vi "Run.vi"(8 "error in (no error)":errorcluster, 10 "Timing Source":string, 11 "Audio Output Queue":refnum<queue>) -> (0 "error out":errorcluster)   [LabVIEW 2019, in "Audio Engine.lvlib"]
doc: "The main audio processing loop.\n\n<b>Priority:</b> Above Normal\n<b>Execution System:</b> Standard"
uses:
  Audio Engine.lvlib
  Audio Output/Audio Output Queue Type.ctl
  <vilib>/Platform/TimedLoop/XDataNode/timing_clust.ctl
  <vilib>/Platform/TimedLoop/XDataNode/nitl_modes.ctl
  <vilib>/Platform/TimedLoop/XDataNode/wakeup.ctl
  Packed Libraries/Globals.lvlibp/Constants.vi
  Packed Libraries/Audio Processing.lvlibp/DBL To I16.vi
  <vilib>/platform/TimedLoop/XDataNode/XDataNode.xnode
  Classes/Deck/Deck.lvclass
  Classes/Mixer/Mixer.lvclass
  <vilib>/Platform/TimedLoop/XDataNode/XDNodeRunTimeDep.lvlib
  Audio Output/Audio Output.lvlib
  Packed Libraries/Globals.lvlibp
  Classes/Effect Unit/Effect Unit.lvclass
  Classes/Channel/Channel.lvclass
  Packed Libraries/Messaging.lvlibp
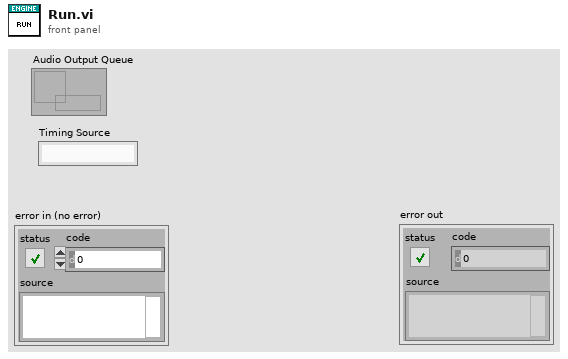
[diagram p1: front panel]
types:
  T1 = typedef "Audio Output.lvlib/Audio Output Queue Type.ctl" = cluster{"Master":waveform(i16)[], "Headphones":waveform(i16)[], "Start Time":dbl}
  T2 = typedef "XDNodeRunTimeDep.lvlib/timing_clust.ctl" = cluster{"Expected End [f-1]":u64, "Actual End [f-1]":u64, "Finished Late? [f-1]":bool, "Expected End [i-1]":u64, "Actual End [i-1]":u64, "Finished Late? [i-1]":bool, "Expected Start [i]":u64, "Actual Start [i]":u64, "Expected Start [f]":u64, "Actual Start [f]":u64, "Source Name":string, "Structure Name":string, "Period":i64, "Deadline":i64, "Offset":i64, "Start":i64, "Priority":i32, "Timeout":i32, "Mode":T3, "Wakeup Reason":T4, "Error":errorcluster, "Source Type":string, "Secondary Source Type":string, "Global End Time":u64, "Global Start Time":u64, "Frame Duration":u64, "Iteration Duration":u64, "Assigned CPU":i32, "I/O Scan Engine Mode":u32}
  T3 = typedef "XDNodeRunTimeDep.lvlib/nitl_modes.ctl" = enum32{"No Change", "Process missed periods, maintain original phase", "Discard missed periods, maintain original phase", "Process missed periods, ignore original phase", "Discard missed periods, ignore original phase"}
  T4 = typedef "XDNodeRunTimeDep.lvlib/wakeup.ctl" = enum32{"Normal", "Aborted", "Asynchronous wakeup", "Timing source error", "Timed loop error", "Timeout"}
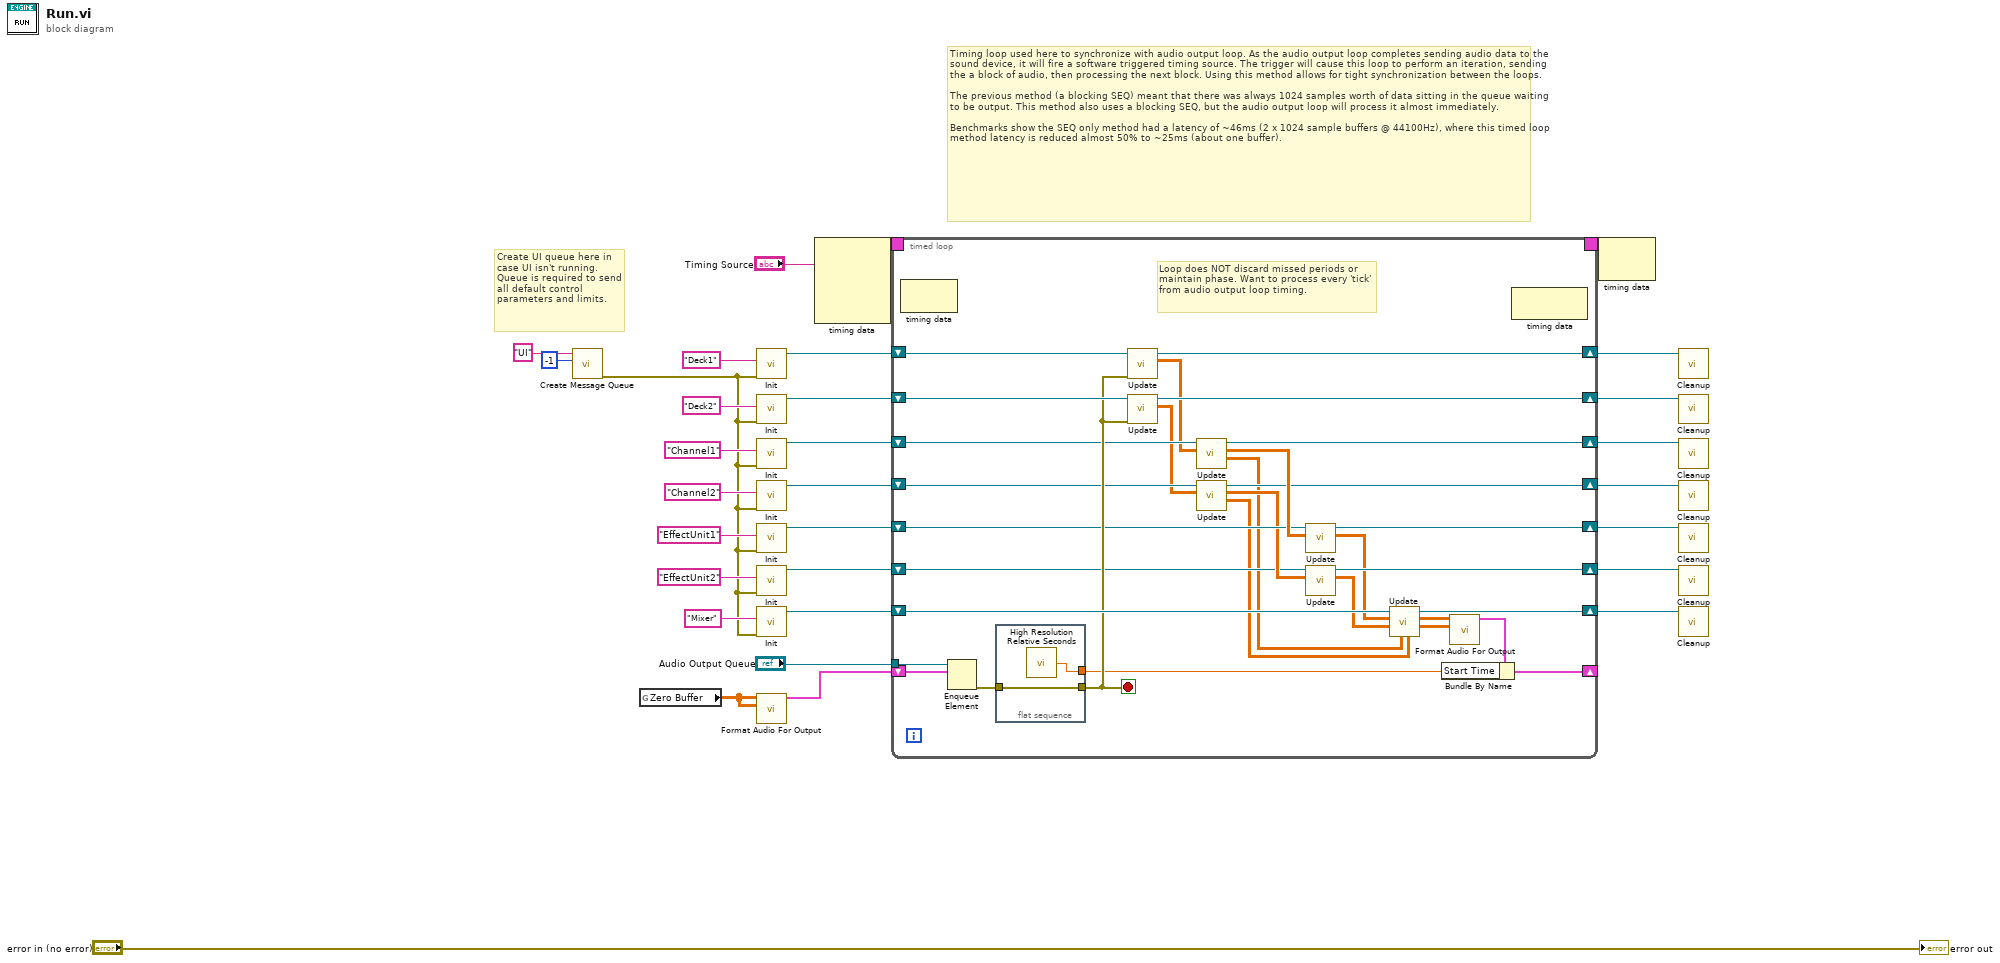
[diagram p0: block diagram]
diagram:
  # "Create UI queue here in case UI isn't running. Queue is required to send all default control parameters and limits."
  # "Timing loop used here to synchronize with audio output loop. As the audio output loop completes sending audio data to the sound device, it will fire a software triggered timing source. The trigger will cause this loop to perform an iteration, sending the a block of audio, then processing the next block. Using this method allows for tight synchronization between the loops.\n\nThe previous method (a blocking SEQ) meant that there was always 1024 samples worth of data sitting in the queue waiting to be output. This method also uses a blocking SEQ, but the audio output loop will process it almost immediately.\n\nBenchmarks show the SEQ only method had a latency of ~46ms (2 x 1024 sample buffers @ 44100Hz), where this timed loop method latency is reduced almost 50% to ~25ms (about one buffer)."
  n1 = call "Create Message Queue.vi"("Max Size (1000)"=-1, "Queue Name"="UI") -> ("error out"=w5:errorcluster)  [unwired: 8 in, 1 out]
  n2 = global read "Constants.vi" "Zero Buffer"() -> (w12:dbl[][])
  n3 = call "Init.vi"("error in (no error)"=w5, "ID"="Deck1") -> ("Deck out"=w29:refnum<class "Deck.lvclass">)  [unwired: 8 in, 1 out]
  n4 = call "Init.vi"("error in (no error)"=w5, "ID"="Deck2") -> ("Deck out"=w28:refnum<class "Deck.lvclass">)  [unwired: 8 in, 1 out]
  n5 = call "Init.vi"("error in (no error)"=w5, "ID"="Channel1") -> ("Channel out"=w19:refnum<class "Channel.lvclass">)  [unwired: 8 in, 1 out]
  n6 = call "Init.vi"("error in (no error)"=w5, "ID"="Channel2") -> ("Channel out"=w18:refnum<class "Channel.lvclass">)  [unwired: 8 in, 1 out]
  n7 = call "Init.vi"("error in (no error)"=w5, "ID"="EffectUnit1") -> ("Effect Unit out"=w21:refnum<class "Effect Unit.lvclass">)  [unwired: 8 in, 1 out]
  n8 = call "Init.vi"("error in (no error)"=w5, "ID"="EffectUnit2") -> ("Effect Unit out"=w20:refnum<class "Effect Unit.lvclass">)  [unwired: 8 in, 1 out]
  n9 = call "Init.vi"("error in (no error)"=w5, "ID"="Mixer") -> ("Mixer out"=w27:refnum<class "Mixer.lvclass">)  [unwired: 8 in, 1 out]
  n10 = call "Format Audio For Output.vi"("Headphone Audio"=w12, "Master Audio"=w12) -> ("Audio Output"=w23:T1)  [unwired: 9 in]
  n11 = node-c288("Timing Source") -> (w7:T2)  [unwired: 3 in]
  n12 = timed-loop {
    shift-right: [w61] -> w26
    shift-left: w29 -> [w62]
    tunnel: "Audio Output Queue" -> [w60]
    shift-right: [w58] -> w25
    shift-left: w28 -> [w59]
    shift-right: [w56] -> w24
    shift-left: w27 -> [w57]
    timing: w7 -> [_]
    timing-out: [_] -> w6
    shift-right: [w48] -> _
    shift-left: w23 -> [w53]
    shift-right: [w36] -> w2
    shift-left: w21 -> [w40]
    shift-right: [w37] -> w1
    shift-left: w20 -> [w38]
    shift-right: [w42] -> w4
    shift-left: w19 -> [w47]
    shift-right: [w41] -> w3
    shift-left: w18 -> [w46]
    stop <- w52 stop-if-true
    # "Loop does NOT discard missed periods or maintain phase. Want to process every 'tick' from audio output loop timing."
    n13 = node-c288() -> ()  [unwired: 1 in, 1 out]
    n14 = Enqueue Element(queue=w60, element=w53) -> (error out=w51:errorcluster)  [unwired: 2 in, 2 out]
    n15 = flat-sequence {
      tunnel: [w64] -> w52
      tunnel: w51 -> [w64]
      tunnel: [w63] -> w50
      frame #0 {
        n16 = call <vilib>:"High Resolution Relative Seconds.vi"() -> ("relative seconds"=w63:dbl)
      }
    }
    n17 = call "Update.vi"("error in (no error)"=w52, "Deck in"=w62) -> ("Audio Block"=w45:dbl[][], "Deck out"=w61:refnum<class "Deck.lvclass">)  [unwired: 7 in, 1 out]
    n18 = call "Update.vi"("error in (no error)"=w52, "Deck in"=w59) -> ("Audio Block"=w44:dbl[][], "Deck out"=w58:refnum<class "Deck.lvclass">)  [unwired: 7 in, 1 out]
    n19 = call "Update.vi"("Audio Block In"=w45, "Channel in"=w47) -> ("Headphones Audio Block Out"=w33:dbl[][], "Master Audio Block Out"=w43:dbl[][], "Channel out"=w42:refnum<class "Channel.lvclass">)  [unwired: 6 in, 1 out]
    n20 = call "Update.vi"("Audio Block In"=w44, "Channel in"=w46) -> ("Headphones Audio Block Out"=w32:dbl[][], "Master Audio Block Out"=w39:dbl[][], "Channel out"=w41:refnum<class "Channel.lvclass">)  [unwired: 6 in, 1 out]
    n21 = call "Update.vi"("Audio Block In"=w43, "Effect Unit in"=w40) -> ("Audio Block Out"=w35:dbl[][], "Effect Unit out"=w36:refnum<class "Effect Unit.lvclass">)  [unwired: 7 in, 1 out]
    n22 = call "Update.vi"("Audio Block In"=w39, "Effect Unit in"=w38) -> ("Audio Block Out"=w34:dbl[][], "Effect Unit out"=w37:refnum<class "Effect Unit.lvclass">)  [unwired: 7 in, 1 out]
    n23 = call "Update.vi"("Headphone Block 2"=w32, "Headphone Block 1"=w33, "Audio Block 2"=w34, "Audio Block 1"=w35, "Mixer in"=w57) -> ("Headphones Audio Block Out"=w54:dbl[][], "Master Audio Block Out"=w55:dbl[][], "Mixer out"=w56:refnum<class "Mixer.lvclass">)  [unwired: 3 in, 1 out]
    n24 = call "Format Audio For Output.vi"("Headphone Audio"=w54, "Master Audio"=w55) -> ("Audio Output"=w49:T1)  [unwired: 9 in]
    n25 = Bundle By Name(cluster=w49, "Start Time"=w50) -> (w48:T1)
    n26 = node-c288() -> ()  [unwired: 1 in, 1 out]
  }
  n27 = node-c288(w6) -> ()  [unwired: 1 out]
  n28 = call "Cleanup.vi"("Deck in"=w26) -> ()  [unwired: 9 in, 2 out]
  n29 = call "Cleanup.vi"("Deck in"=w25) -> ()  [unwired: 9 in, 2 out]
  n30 = call "Cleanup.vi"("Channel in"=w4) -> ()  [unwired: 10 in, 1 out]
  n31 = call "Cleanup.vi"("Channel in"=w3) -> ()  [unwired: 10 in, 1 out]
  n32 = call "Cleanup.vi"("Effect Unit in"=w2) -> ()  [unwired: 9 in, 2 out]
  n33 = call "Cleanup.vi"("Effect Unit in"=w1) -> ()  [unwired: 9 in, 2 out]
  n34 = call "Cleanup.vi"("Mixer in"=w24) -> ()  [unwired: 10 in, 1 out]
  "error out" <- "error in (no error)"
